vi "Write U32.vi"(7 "RegisterOffset":u32, 8 "error in":errorcluster, 9 "value in":u32, 10 "register name":string, 11 "session in":u32) -> (0 "error out":errorcluster, 3 "session out":u32)   [LabVIEW 2020, in "FPGA Register IO.lvlib"]
uses:
  FPGA Register IO.lvlib
  NiFpga.dll
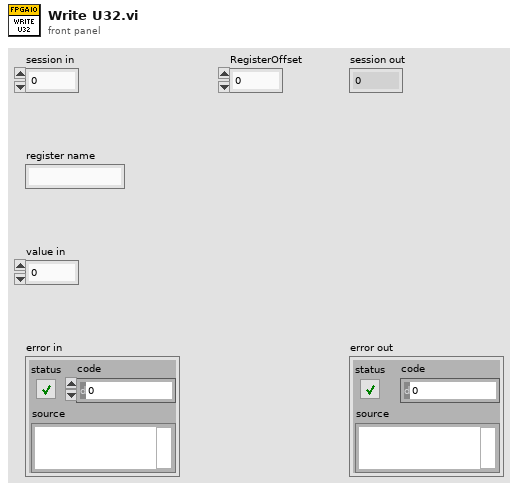
[diagram p1: front panel]
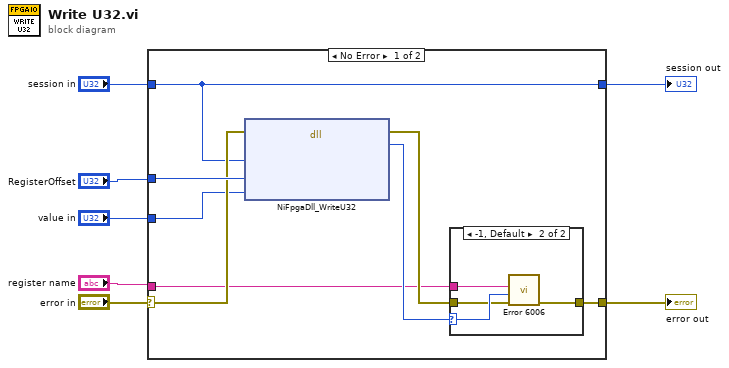
[diagram p0: block diagram]
diagram:
  n1 = case shown="No Error" "error in" {
    selector: "error in" -> [w14 w22]
    tunnel: "session in" -> [w13 w21]
    tunnel: [w11 w22] -> w6
    tunnel: "RegisterOffset" -> [w15 _]
    tunnel: [w13 w21] -> w5
    tunnel: "value in" -> [w12 _]
    tunnel: "register name" -> [w8 _]
    frame No Error {
      n2 = dll-call lib="NiFpga.*" fn="NiFpgaDll_WriteU32"(error in=w14, "session"=w13, "offset"=w15, "value"=w12) -> (error out=w9:errorcluster, "status"=w10:i32)  [unwired: 5 in, 1 out]
      n3 = case shown="-1, Default" w10 {
        selector: w10 -> [_ w18]
        tunnel: w9 -> [w16 w17]
        tunnel: [w16 w20] -> w11
        tunnel: w8 -> [_ w19]
        frame 0 {
        }
        frame -1, Default {
          n4 = call "Error 6006.vi"("error in (no error)"=w17, "rio status code"=w18, "register name"=w19) -> ("error out"=w20:errorcluster)  [unwired: 8 in]
        }
      }
    }
    frame Error {
    }
  }
  "error out" <- w6
  "session out" <- w5
